vi "CustomizeMenubar.vi"(8 "error in (no error)":errorcluster, 10 "remove file close?":bool, 11 "menubar":refnum<k9>) -> (0 "error out":errorcluster)   [LabVIEW 2023, in "GettingStartedWindow.lvlib"]
uses:
  <resource>/modes/FRC/GSW/GettingStartedWindow.lvlib
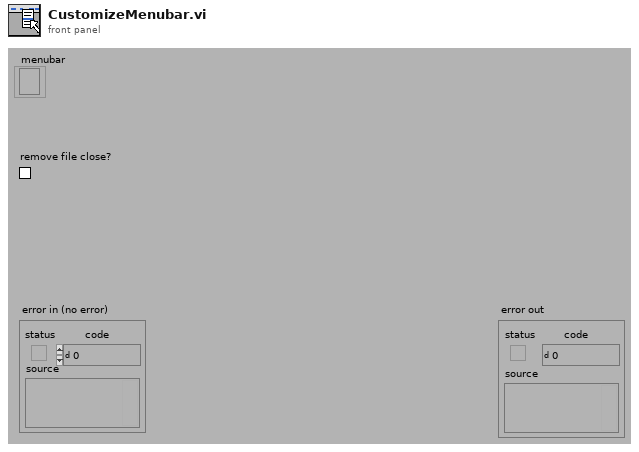
[diagram p1: front panel]
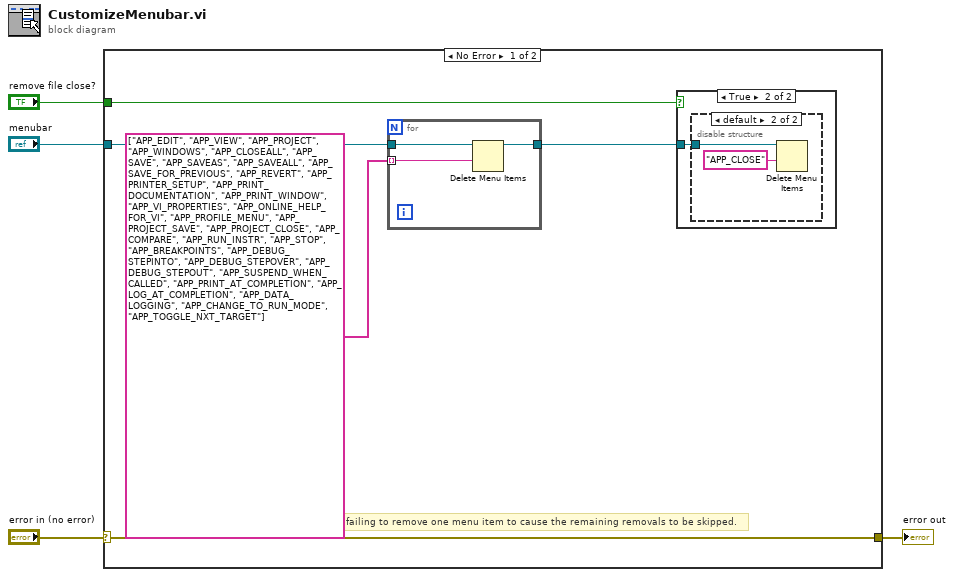
[diagram p0: block diagram]
diagram:
  n1 = case shown="No Error" "error in (no error)" {
    selector: "error in (no error)" -> [w7 w16]
    tunnel: [w7 w16] -> w3
    tunnel: "menubar" -> [w6 _]
    tunnel: "remove file close?" -> [w5 _]
    frame No Error {
      # "Intentionally ignoring errors - we don't want failing to remove one menu item to cause the remaining removals to be skipped."
      n2 = for {
        tunnel: w6 -> [w12]
        tunnel: [w11] -> w9
        tunnel: string[] ["APP_EDIT", "APP_VIEW", "APP_PROJECT", "APP_WINDOWS", "APP_CLOSEALL", "APP_SAVE", "APP_SAVEAS", "APP_SAVEALL", "APP_SAVE_FOR_PREVIOUS", "APP_REVERT", "APP_PRINTER_SETUP", "APP_PRINT_DOCUMENTATION", "APP_PRINT_WINDOW", "APP_VI_PROPERTIES", "APP_ONLINE_HELP_FOR_VI", "APP_PROFILE_MENU", "APP_PROJECT_SAVE", "APP_PROJECT_CLOSE", "APP_COMPARE", "APP_RUN_INSTR", "APP_STOP", "APP_BREAKPOINTS", "APP_DEBUG_STEPINTO", "APP_DEBUG_STEPOVER", "APP_DEBUG_STEPOUT", "APP_SUSPEND_WHEN_CALLED", "APP_PRINT_AT_COMPLETION", "APP_LOG_AT_COMPLETION", "APP_DATA_LOGGING", "APP_CHANGE_TO_RUN_MODE", "APP_TOGGLE_NXT_TARGET"] -> [w10] mode=indexing
        n3 = Delete Menu Items(7:w10, 9:w12) -> (3:w11:refnum<k9>)  [unwired: 1 in, 2 out]
      }
      n4 = case shown="True" w5 {
        tunnel: w9 -> [_ w13]
        frame False {
        }
        frame True {
          n5 = disable-structure "Conditional Disable Structure" shown="default" {
            disable-tunnel: w13 -> [_ w15]
            frame condition #0 {
              # "Mac always has\nFile>Close enabled\nbecause it doesn't\nmake us exit \nLabVIEW."
            }
            frame condition #1 (active) {
              n6 = Delete Menu Items(7:"APP_CLOSE" ("items"), 9:w15) -> ()  [unwired: 1 in, 3 out]
            }
          }
        }
      }
    }
    frame Error {
    }
  }
  "error out" <- w3
